vi "Parse INI File.vi"(8 "error in (no error)":errorcluster, 11 "File Path":path) -> (0 "error out":errorcluster, 1 "Values":string[](array[string]), 2 "Keys":string[](array[string]), 3 "Sections":string[](array[string]))   [LabVIEW 2024]
doc: "Reads an INI file and returns every key = value line as three parallel arrays: the section the key is in, the key name, and the value. A value in double quotes is returned without the quotes, with the escapes \\\\, \\0A and \\0D turned back into a backslash, a line feed and a carriage return; an unquoted value (TRUE, FALSE, a number) is returned as written. Blank lines, comment lines and lines without = are skipped. A file that does not exist returns empty arrays and no error.\n\nThis is a plain text parser on purpose: it reads the schema-version-2 files and the old version-1 files alike, and needs no configuration-file refnum.\n\nGenerated by: Claude"
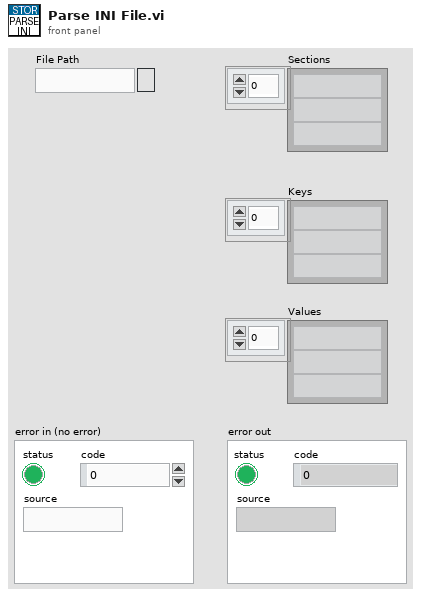
[diagram p1: front panel]
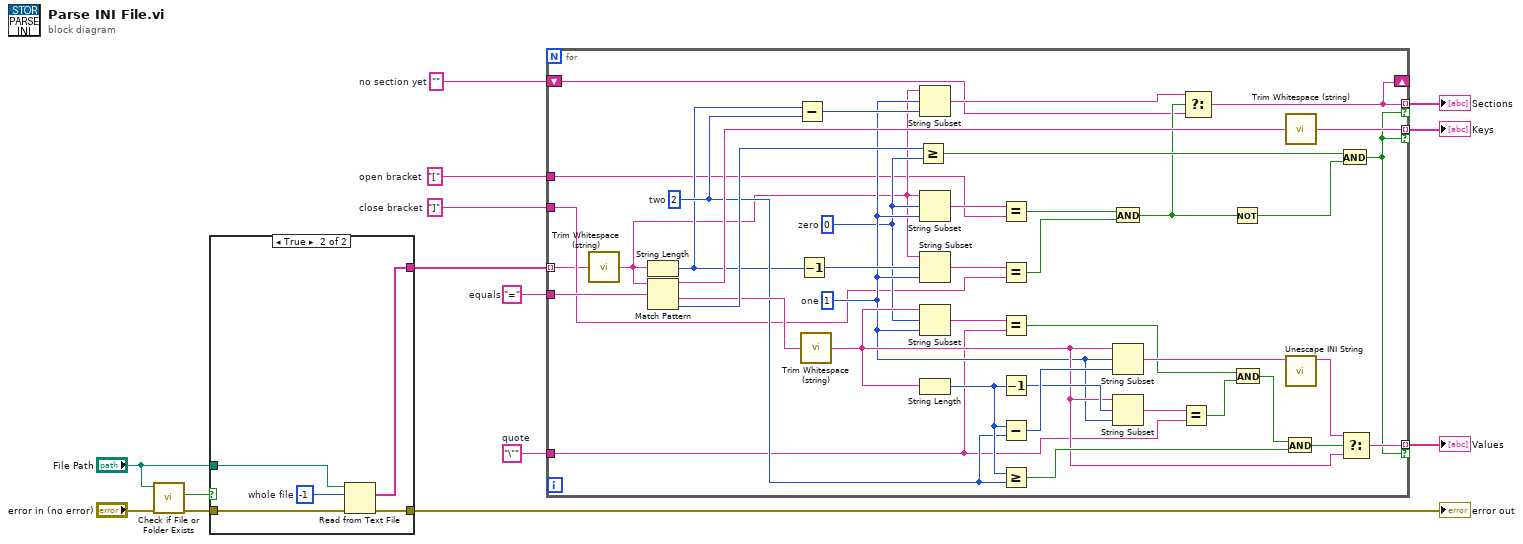
[diagram p0: block diagram]
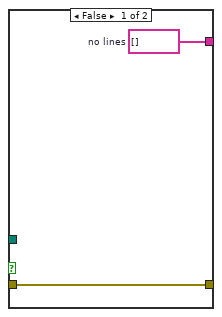
[diagram p2: hidden frame]
diagram:
  w11 = "\""  # quote
  w10 = "="  # equals
  w9 = "]"  # close bracket
  w8 = "["  # open bracket
  w7 = ""  # no section yet
  n1 = call <vilib>:"Check if File or Folder Exists.vi"("error in (no error)"="error in (no error)", "path"="File Path") -> ("error out"=w3:errorcluster, "file or folder exists?"=w4:bool)  [unwired: 7 in, 1 out]
  n2 = case shown="True" w4 {
    tunnel: "File Path" -> [_ w17]
    tunnel: [w16 w20] -> w5
    tunnel: w3 -> [w15 w18]
    tunnel: [w15 w21] -> w6
    frame False {
      w16 = string[] []  # no lines
    }
    frame True {
      w19 = -1  # whole file
      n3 = Read from Text File(file (use dialog)=w17, count=w19, error in=w18) -> (text=w20:string[], error out=w21:errorcluster)  [unwired: 1 in, 2 out]
    }
  }
  "error out" <- w6
  n4 = for {
    tunnel: w8 -> [w23]
    tunnel: w9 -> [w24]
    tunnel: w10 -> [w25]
    tunnel: w11 -> [w26]
    shift-right: [w28] -> _
    shift-left: w7 -> [w27]
    tunnel: w5 -> [w22] mode=indexing
    tunnel: [w48] -> w13 mode=indexing if=w47
    tunnel: [w28] -> w12 mode=indexing if=w47
    tunnel: [w62] -> w14 mode=indexing if=w47
    w33 = 2  # two
    w32 = 1  # one
    w31 = 0  # zero
    n5 = call <vilib>:"Trim Whitespace (string).vi"("string"=w22) -> ("trimmed string"=w29:string)  [unwired: 1 in]
    n6 = String Length(string=w29) -> (length=w30:i32)
    n7 = Match Pattern(string=w29, regular expression=w25) -> (before substring=w42:string, after substring=w43:string, offset past match=w44:i32)  [unwired: 1 in, 1 out]
    n8 = Subtract(x=w30, y=w33) -> (x-y=w40:i32)
    n9 = Decrement(x=w30) -> (x-1=w35:i32)
    n10 = call <vilib>:"Trim Whitespace (string).vi"("string"=w43) -> ("trimmed string"=w49:string)  [unwired: 1 in]
    n11 = Greater Or Equal?(x=w44, y=w31) -> (x >= y?=w45:bool)
    n12 = String Subset(string=w29, offset (0)=w32, length (rest)=w40) -> (substring=w41:string)
    n13 = String Subset(string=w29, offset (0)=w31, length (rest)=w32) -> (substring=w34:string)
    n14 = String Subset(string=w29, offset (0)=w35, length (rest)=w32) -> (substring=w36:string)
    n15 = String Subset(string=w49, offset (0)=w31, length (rest)=w32) -> (substring=w51:string)
    n16 = String Length(string=w49) -> (length=w50:i32)
    n17 = Equal?(x=w34, y=w23) -> (x = y?=w37:bool)
    n18 = Equal?(x=w36, y=w24) -> (x = y?=w38:bool)
    n19 = Equal?(x=w51, y=w26) -> (x = y?=w54:bool)
    n20 = Decrement(x=w50) -> (x-1=w52:i32)
    n21 = Subtract(x=w50, y=w33) -> (x-y=w59:i32)
    n22 = Greater Or Equal?(x=w50, y=w33) -> (x >= y?=w56:bool)
    n23 = And(x=w37, y=w38) -> (x .and. y?=w39:bool)
    n24 = String Subset(string=w49, offset (0)=w32, length (rest)=w59) -> (substring=w60:string)
    n25 = String Subset(string=w49, offset (0)=w52, length (rest)=w32) -> (substring=w53:string)
    n26 = Equal?(x=w53, y=w26) -> (x = y?=w55:bool)
    n27 = Select(t=w41, s=w39, f=w27) -> (s? t:f=w28:string)
    n28 = Not(x=w39) -> (.not. x?=w46:bool)
    n29 = And(x=w54, y=w55) -> (x .and. y?=w57:bool)
    n30 = And(x=w57, y=w56) -> (x .and. y?=w58:bool)
    n31 = call <vilib>:"Trim Whitespace (string).vi"("string"=w42) -> ("trimmed string"=w48:string)  [unwired: 1 in]
    n32 = call "Unescape INI String.vi"("Escaped"=w60) -> ("Text"=w61:string)  [unwired: 9 in, 1 out]
    n33 = And(x=w45, y=w46) -> (x .and. y?=w47:bool)
    n34 = Select(t=w61, s=w58, f=w49) -> (s? t:f=w62:string)
  }
  "Sections" <- w12
  "Keys" <- w13
  "Values" <- w14
